vi "Filter Options.vi"(10 "Text":string, 11 "All Options":string[](array[string])) -> (3 "Filtered Names":string[](array[string]))   [LabVIEW 2020, in "AutoComplete.lvlib"]
uses:
  AutoComplete.lvlib
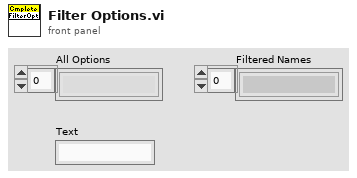
[diagram p1: front panel]
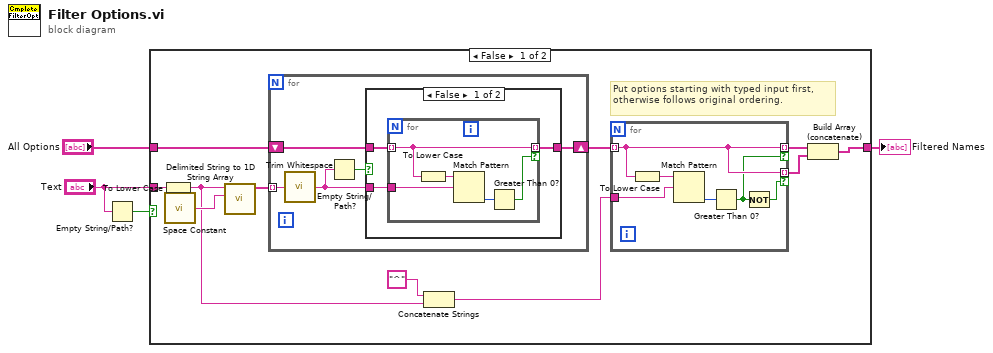
[diagram p0: block diagram]
diagram:
  n1 = Empty String/Path?(string/path="Text") -> (empty?=w3:bool)
  n2 = case shown="False" w3 {
    tunnel: [w5 w36] -> w1
    tunnel: "All Options" -> [w15 w36]
    tunnel: "Text" -> [w14 _]
    frame False {
      # "Put options starting with typed input first, otherwise follows original ordering."
      n3 = To Lower Case(string=w14) -> (all lower case string=w10:string)
      n4 = call <vilib>:"Space Constant.vi"() -> ("String"=w13:string)
      n5 = call <vilib>:"Delimited String to 1D String Array.vi"("delimiter"=w13, "delimited string"=w10) -> ("string array"=w12:string[])  [unwired: 9 in]
      n6 = for {
        shift-right: [w26] -> w9
        shift-left: w15 -> [w25]
        tunnel: w12 -> [w24] mode=indexing
        n7 = call <vilib>:"Trim Whitespace.vi"("string"=w24) -> ("trimmed string"=w23:string)  [unwired: 1 in]
        n8 = Empty String/Path?(string/path=w23) -> (empty?=w22:bool)
        n9 = case shown="False" w22 {
          tunnel: [w29 w35] -> w26
          tunnel: w25 -> [w28 w35]
          tunnel: w23 -> [w27 _]
          frame False {
            n10 = for {
              tunnel: w27 -> [w32]
              tunnel: [w31] -> w29 mode=indexing if=w33
              tunnel: w28 -> [w31] mode=indexing
              n11 = To Lower Case(string=w31) -> (all lower case string=w30:string)
              n12 = Match Pattern(string=w30, regular expression=w32) -> (offset past match=w34:i32)  [unwired: 1 in, 3 out]
              n13 = Greater Than 0?(x=w34) -> (x > 0?=w33:bool)
            }
          }
          frame True {
          }
        }
      }
      n14 = Concatenate Strings("^" ("string"), w10) -> (w8:string)
      n15 = for {
        tunnel: w9 -> [w18] mode=indexing
        tunnel: w8 -> [w20]
        tunnel: [w18] -> w7 mode=indexing if=w16
        tunnel: [w18] -> w6 mode=indexing if=w17
        n16 = To Lower Case(string=w18) -> (all lower case string=w21:string)
        n17 = Match Pattern(string=w21, regular expression=w20) -> (offset past match=w19:i32)  [unwired: 1 in, 3 out]
        n18 = Greater Than 0?(x=w19) -> (x > 0?=w16:bool)
        n19 = Not(x=w16) -> (.not. x?=w17:bool)
      }
      n20 = Build Array (concatenate)(w7, w6) -> (w5:string[])
    }
    frame True {
    }
  }
  "Filtered Names" <- w1
